vi "RFH-add-Permittivity_from_calc2.vi"() -> ()   [LabVIEW 2020, in "RFH-Reflection_File_Handler.lvlib"]
doc: "Run by hand: reads the files of a data folder, computes the permittivity with the Bilinear method from the chosen air/open, DI water and salt water files, and saves the results. The user picks the folder, the standards and the water temperature."
uses:
  RFH-Reflection_File_Handler.lvlib
  Computation/RDC-Reflection_Data_Computation.lvlib
panel:
  in  "Add Ideal Perm?":bool
  out "Array of file paths":path[](array[path])
  in  "Salt water":path=path "C:/projects/Universitet/Master/data/Simulated data/Saltwater/complete/100M/sim-P1-saltwater-22p5c.s2p"
  in  "Di water":path=path "C:/projects/Universitet/Master/data/Simulated data/Water/complete/100M/sim-P1-DI_water-22p5c.s2p"
  in  "air/open":path=path "C:/projects/Universitet/Master/data/Simulated data/Other/complete/100M/sim-P1-open.s2p"
  in  "Data source dir":path=path "C:/projects/Universitet/Master/data/autopermtest/lib"
  in  "water Temp (22.5C) [10-40C]":dbl=22.5
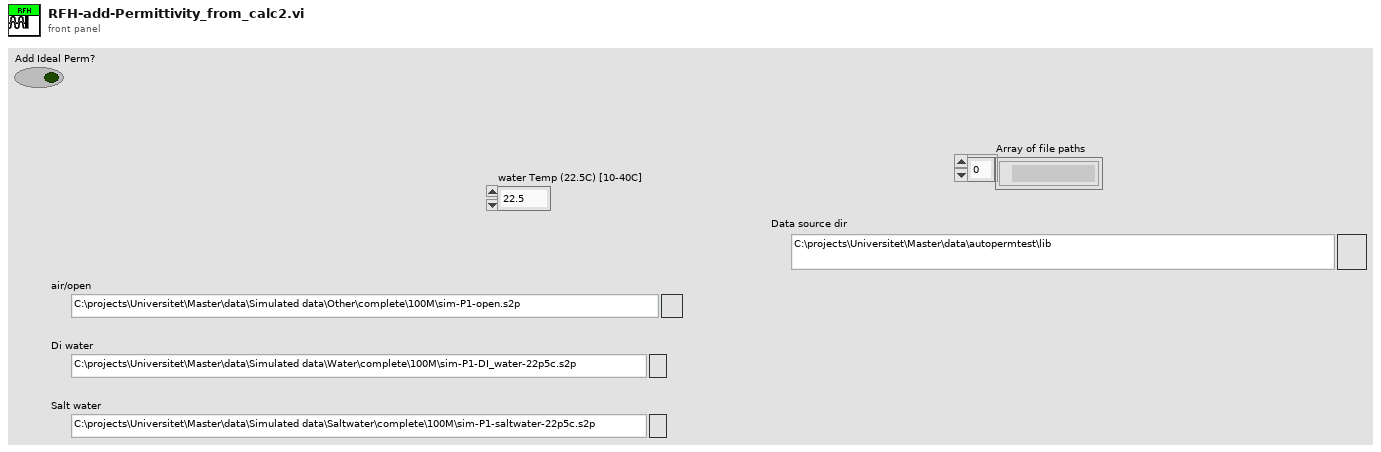
[diagram p1: front panel]
types:
  T1 = typedef "RFH-Reflection_File_Handler.lvlib/RFH-common_data_format.ctl" = cluster{"Frequency":dbl[], "Reflection'":dbl[], "Reflection''":dbl[], "Permativity'":dbl[], "Permativity''":dbl[], "Conductivity":dbl[], "Loss Tangent":dbl[], "Resistance":dbl[], "Reactance":dbl[]}
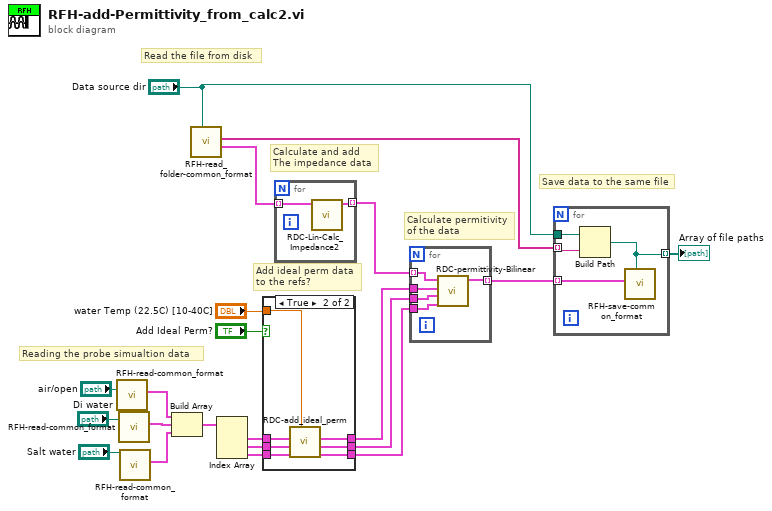
[diagram p0: block diagram]
diagram:
  # "Reading the probe simualtion data"
  # "Read the file from disk"
  # "Calculate and add\nThe impedance data"
  # "Save data to the same file"
  # "Calculate permitivity \nof the data"
  # "Add ideal perm data\nto the refs?"
  n1 = call "RFH-read-common_format.vi"("file path (dialog if empty)"="air/open") -> ("Common Format"=w17:T1)  [unwired: 9 in, 1 out]
  n2 = call "RFH-read-common_format.vi"("file path (dialog if empty)"="Di water") -> ("Common Format"=w16:T1)  [unwired: 9 in, 1 out]
  n3 = call "RFH-read-common_format.vi"("file path (dialog if empty)"="Salt water") -> ("Common Format"=w15:T1)  [unwired: 9 in, 1 out]
  n4 = Build Array(w17, w16, w15) -> (w14:T1[])
  n5 = call "RFH-read_folder-common_format.vi"("File Path"="Data source dir") -> ("Data"=w4:T1[], "Names"=w1:string[])  [unwired: 8 in, 1 out]
  n6 = Index Array(array=w14) -> (element #1=w13:T1, element #2=w12:T1, element #3=w11:T1)  [unwired: 3 in]
  n7 = case shown="True" "Add Ideal Perm?" {
    tunnel: w13 -> [w24 w31]
    tunnel: w12 -> [w23 w30]
    tunnel: w11 -> [w22 w29]
    tunnel: [w24 w28] -> w9
    tunnel: [w23 w27] -> w8
    tunnel: [w22 w26] -> w7
    tunnel: "water Temp (22.5C) [10-40C]" -> [_ w25]
    frame False {
    }
    frame True {
      n8 = call "RDC-add_ideal_perm.vi"("water Temp (25C) [10-40C]"=w25, "Salt Water"=w29, "DI-Water"=w30, "Open/Air"=w31) -> ("Salt Water out"=w26:T1, "DI-Water  out"=w27:T1, "Open/Air out"=w28:T1)  [unwired: 5 in]
    }
  }
  n9 = for {
    tunnel: w4 -> [w33] mode=indexing
    tunnel: [w32] -> w3 mode=indexing
    n10 = call "RDC-Lin-Calc_Impedance2.vi"("input cluster"=w33) -> ("Output cluster"=w32:T1)  [unwired: 9 in, 1 out]
  }
  n11 = for {
    tunnel: w9 -> [w38]
    tunnel: w8 -> [w37]
    tunnel: w7 -> [w36]
    tunnel: w3 -> [w35] mode=indexing
    tunnel: [w34] -> w10 mode=indexing
    n12 = call "RDC-permittivity-Bilinear.vi"("Salt Water"=w36, "DI-Water"=w37, "Open/Air"=w38, "Common Format"=w35) -> ("Common Format out"=w34:T1)  [unwired: 7 in]
  }
  n13 = for {
    tunnel: "Data source dir" -> [w42]
    tunnel: w1 -> [w41] mode=indexing
    tunnel: w10 -> [w39] mode=indexing
    tunnel: [w40] -> w5 mode=indexing
    n14 = Build Path(base path=w42, name or relative path=w41) -> (appended path=w40:path)
    n15 = call "RFH-save-common_format.vi"("file path (use dialog)"=w40, "Common Format"=w39) -> ()  [unwired: 9 in, 1 out]
  }
  "Array of file paths" <- w5
